vi "Sous_VI_Avancer.vi"(8 "error in (no error)":errorcluster, 11 "Énum":enum16{"Droite", "Gauche"}(ring)=enum."Gauche") -> (0 "error out":errorcluster, 3 "Info de fin de Parcours":bool, 5 "Détection ligne":bool[](array[boolean]))   [LabVIEW 2018]
doc: "Avance jusqu'à atteindre une ligne à droite/gauche"
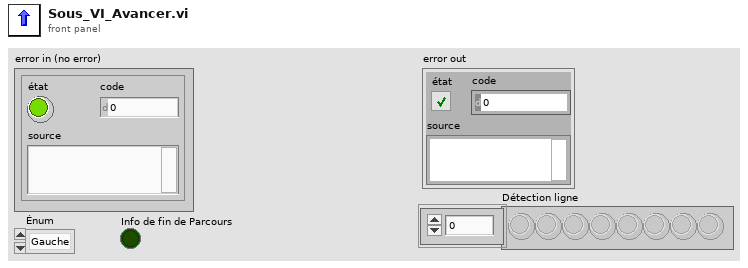
[diagram p1: front panel]
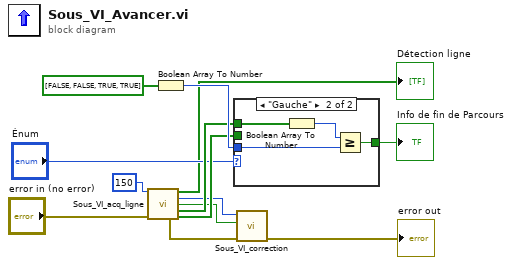
[diagram p0: block diagram]
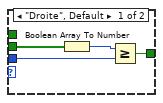
[diagram p2: hidden frame]
diagram:
  n1 = call "Sous_VI_acq_ligne.vi"("Seuil"=150, "error in (no error)"="error in (no error)") -> ("x > y ?"=→"Détection ligne":bool[], "Décalage"=w8:u32, "G/D ?"=w7:bool, "4 LED gauches"=w10:bool[], "error out"=w13:errorcluster, "4 LED droite"=w9:bool[])  [unwired: 8 in]
  n2 = Boolean Array To Number(Boolean array=bool[] [FALSE, FALSE, TRUE, TRUE] ("x < y ? 2")) -> (number=w12:u32)
  n3 = case shown="\"Gauche\"" "Énum" {
    tunnel: w9 -> [w16 _]
    tunnel: w10 -> [_ w20]
    tunnel: [w15 w19] -> w2
    tunnel: w12 -> [w14 w18]
    frame "Droite", Default {
      n4 = Boolean Array To Number(Boolean array=w16) -> (number=w17:u32)
      n5 = Greater Or Equal?(x=w17, y=w14) -> (x >= y?=w15:bool)
    }
    frame "Gauche" {
      n6 = Boolean Array To Number(Boolean array=w20) -> (number=w21:u32)
      n7 = Greater Or Equal?(x=w21, y=w18) -> (x >= y?=w19:bool)
    }
  }
  "Info de fin de Parcours" <- w2
  n8 = call "Sous_VI_correction.vi"("error in (no error)"=w13, "G/D ?"=w7, "Décalage"=w8) -> ("error out"=→"error out":errorcluster)  [unwired: 8 in]
